vi "Dual Camera Control.vi"(7 "Calling VI Ref":refnum<vi>) -> ()   [LabVIEW 2016]
uses:
  Hardware Configuration/Hardware Configuration Controls/Device Function.ctl
  Dual Camera Control Type Defs/Dual Camera Notifier Type.ctl
  Dual Camera Control Type Defs/Dual Camera Actions.ctl
  <vilib>/Utility/miscctls.llb/LVPointTypeDef.ctl
  Device Library/Cameras/Camera Controls/Generic Camera Actions.ctl
  <vilib>/vision/Image Controls.llb/IMAQ Image.ctl
  Device Library/Cameras/Camera Controls/Generic Camera ROI.ctl
  Hardware Configuration/Hardware Configuration Controls/Device Type.ctl
  Laser Control/Laser Power Control/Laser Power Control Type Defs/Laser Power Ctrl Messenger Actions.ctl
  <vilib>/Utility/error.llb/whitespace.ctl
  shell32.dll
panel:
  in  "Capture":bool
  in  "Preview":bool
  in  "Quit":bool
  out "Current Frame":u32=1
  in  "Exposure Time (s)":dbl=0.1
  in  "Base Save Path":path
  in  "File Name":string="Test Image"
  in  "Number of Frames":u32=1
  in  "Camera 02":bool=TRUE
  in  "Camera 01":bool=TRUE
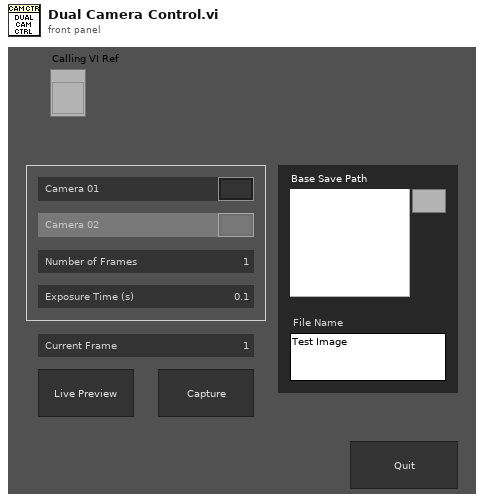
[diagram p1: front panel]
types:
  T1 = typedef "Generic Camera Actions.ctl" = enum16{"Status", "Live Preview", "Capture", "Abort", "Set Exposure Time (s)", "Get Exposure Time (s)", "Record Settings", "Binning", "Set ROI", "Get ROI", "Defect Correction On?", "Cooler On?", "Fan On?", "Quit"}
  T2 = typedef "Generic Camera ROI.ctl" = cluster{"H_Offset":u16, "V_Offset":u16, "H_Width":u16, "V_Width":u16}
  T3 = typedef "IMAQ Image.ctl" = refnum<image>
  T4 = enum16{"Always On", "Always Off", "Off While Running"}
  T5 = typedef "LVPointTypeDef.ctl" = cluster{"Horizontal":i16, "Vertical":i16}
  T6 = typedef "Dual Camera Actions.ctl" = enum16{"Idle", "Exposure Time", "Preview", "Capture", "Set Save Path", "Lasers On", "Lasers Off", "Start Acquisition", "Abort", "Exit Loop", "Quit"}
  T7 = typedef "Dual Camera Notifier Type.ctl" = cluster{"Actions":T6, "Exposure Time (s)":dbl, "Num of Frames":u32, "Save Path":path, "Running?":bool, "Active Cameras":bool[]}
  T8 = typedef "Device Function.ctl" = enum16{"Primary", "Secondary", "Overview", "Wide Field Drift Correction", "642 nm Excitation", "560 nm Excitation", "940 nm Excitation", "546 nm Excitation", "488 nm Excitation", "405 nm Excitation", "Objective Drift Correction", "4Pi Objective Lock", "Objective XY", "Objective Z", "Sample XY", "Sample Coarse Z", "Sample Z", "4Pi Lower", "4Pi Upper", "Mojo", "Adj Cavity", "Line Scanning", "Alert"}
  T9 = enum8{"Enabled", "Disabled", "Disabled and Grayed Out"}
  T10 = typedef "Device Type.ctl" = enum16{"AOTF", "Camera", "Deformable Mirror", "Laser", "Shutter", "Stage", "Waveform", "FPGA", "Email", "Filter Wheel"}
  T11 = typedef "LVRectTypeDef.ctl" = cluster{"Left":i16, "Top":i16, "Right":i16, "Bottom":i16}
  T12 = typedef "LVBoundsTypeDef.ctl" = cluster{"Width":u32, "Height":u32}
  T13 = typedef "Image Type" = u32
  T14 = typedef "whitespace.ctl" = u16
  T15 = typedef "Laser Power Ctrl Messenger Actions.ctl" = enum16{"All Active On", "All Off", "Adjust Power", "Line On/Off", "Get Status"}
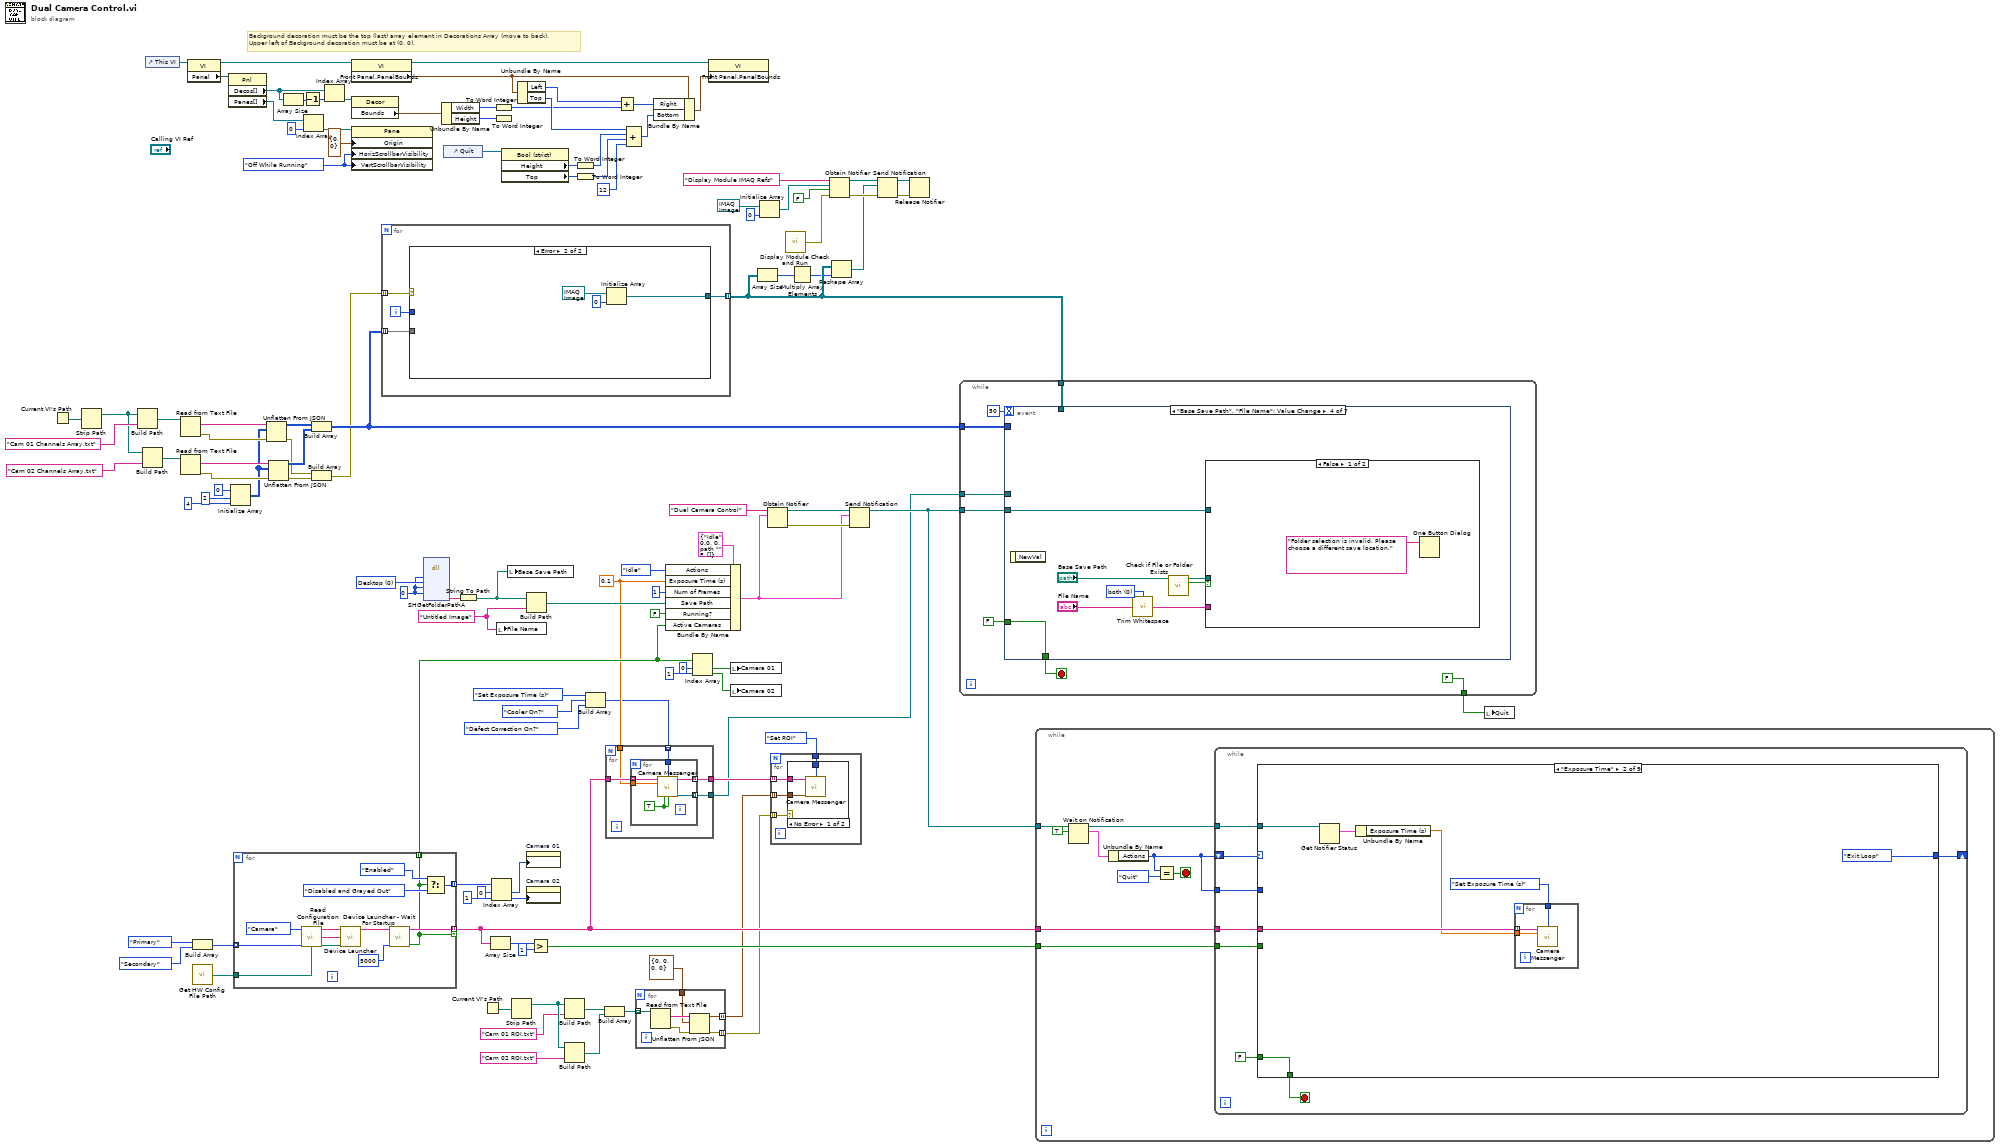
[diagram p0: block diagram]
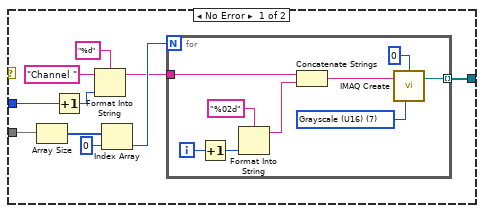
[diagram p3: hidden frame]
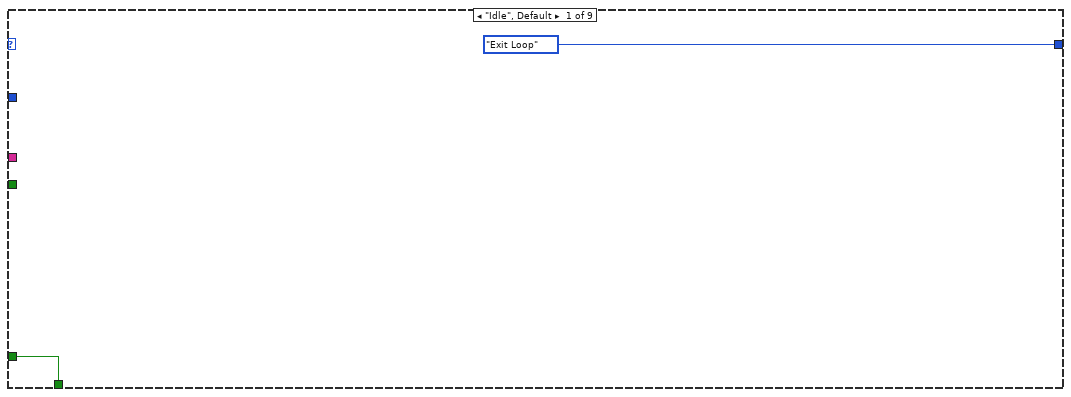
[diagram p4: hidden frame]
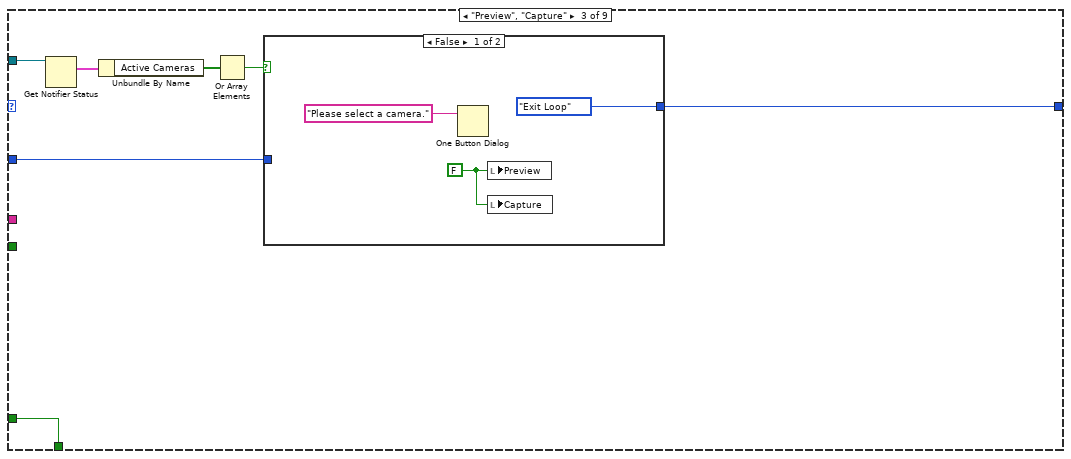
[diagram p5: hidden frame]
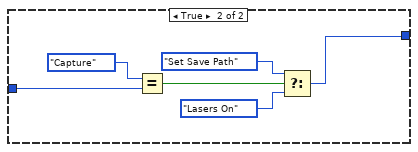
[diagram p6: hidden frame]
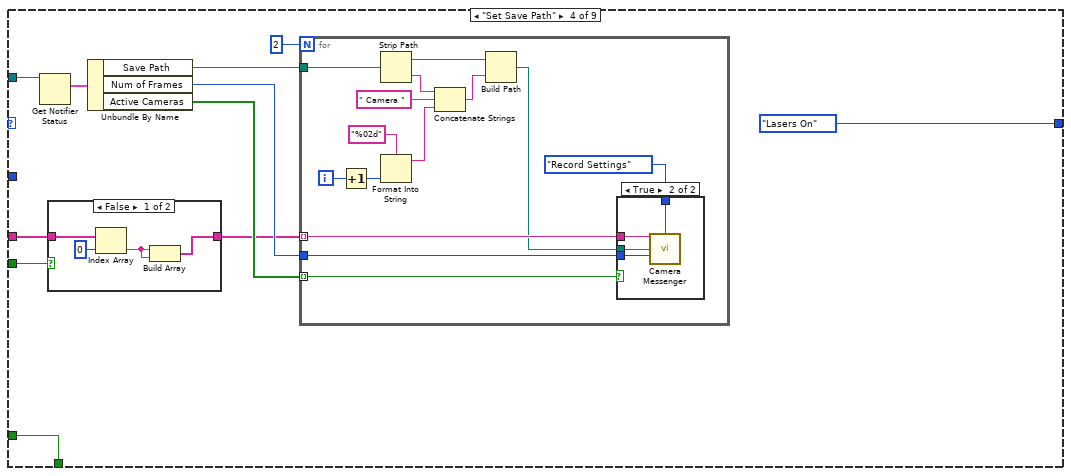
[diagram p7: hidden frame]
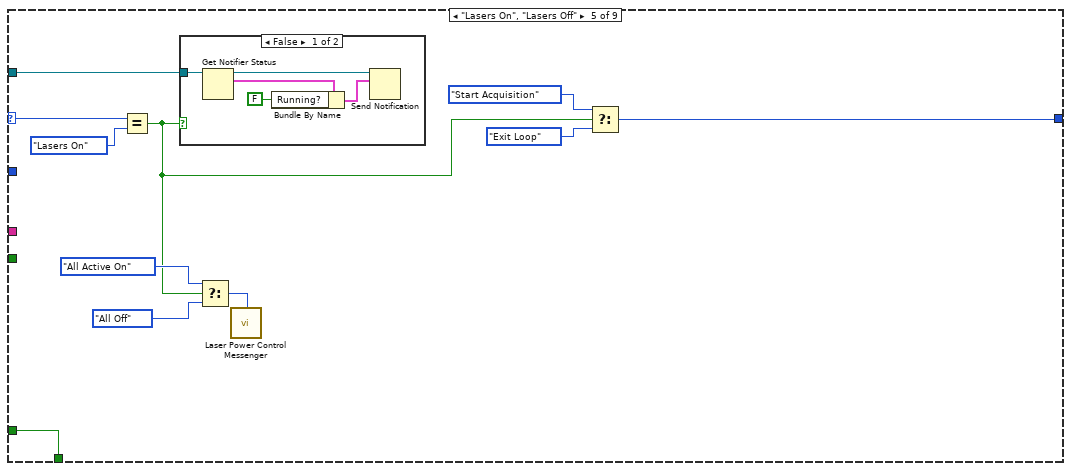
[diagram p10: hidden frame]
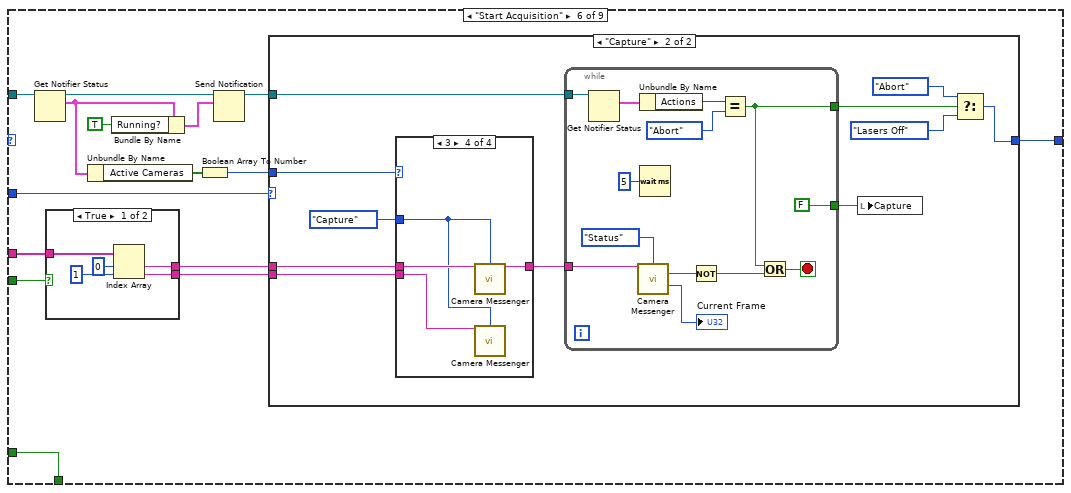
[diagram p12: hidden frame]
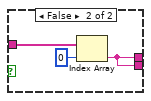
[diagram p13: hidden frame]
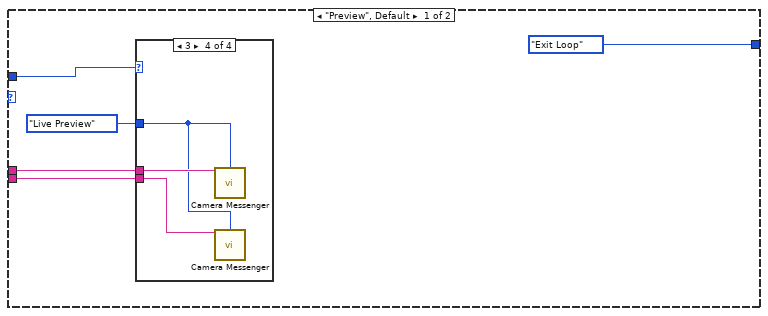
[diagram p14: hidden frame]
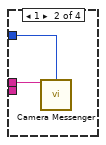
[diagram p16: hidden frame]
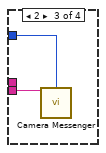
[diagram p17: hidden frame]
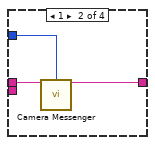
[diagram p19: hidden frame]
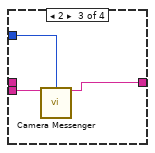
[diagram p20: hidden frame]
diagram:
  w65 = T4."Off While Running" ("Vertical Scrollbar Visibility")
  w39 = 0.1 ("Exposure Time (s)")
  w108 = "Untitled Image"
  w111 = 0 items=["Desktop"=0, "Personal Documents"=5, "AppData"=26, "Local AppData"=28, "Common AppData"=35, "Program Files"=38, "Program Files Common"=43, "Common Documents"=46] ("Requested Path")
  w110 = 0 ("HWND")
  # "Background decoration must be the top (last) array element in Decorations Array (move to back).\nUpper left of Background decoration must be at (0, 0)."
  n1 = Current VI's Path() -> (path=w49:path)
  n2 = Strip Path(path=w49) -> (stripped path=w48:path)  [unwired: 1 out]
  n3 = Build Path(base path=w48, name or relative path="Cam 01 Channels Array.txt") -> (appended path=w52:path)
  n4 = Build Path(base path=w48, name or relative path="Cam 02 Channels Array.txt") -> (appended path=w42:path)
  n5 = control-ref of="This VI"() -> (w57:refnum<vi>)
  n6 = Read from Text File(file (use dialog)=w52) -> (text=w51:string, error out=w50:errorcluster)  [unwired: 3 in, 2 out]
  n7 = Read from Text File(file (use dialog)=w42) -> (text=w45:string, error out=w46:errorcluster)  [unwired: 3 in, 2 out]
  n8 = property class="VI"(reference=w57) -> (reference out=w66:refnum<vi>, "Panel"=w58:refnum<vi>)  [unwired: 1 in, 1 out]
  n9 = Build Array(Device_Function."Primary" ("Device Function"), Device_Function."Secondary" ("Device Function")) -> (w113:T8[])
  n10 = call "Get HW Config File Path.vi"() -> ("File Path"=w96:path)  [unwired: 14 in, 1 out]
  n11 = property class="Pnl"(reference=w58) -> ("Decos[]"=w56:refnum<vi>[], "Panes[]"=w62:refnum<vi>[])  [unwired: 1 in, 2 out]
  n12 = Initialize Array(0 ("element"), 2 ("dimension size"), 4 ("dimension size")) -> (w41:i32[][])
  n13 = for {
    tunnel: w113 -> [w124] mode=indexing
    tunnel: w96 -> [w123]
    tunnel: [w121] -> w40 mode=indexing if=w116
    tunnel: [w117] -> w95 mode=indexing
    tunnel: [w116] -> w87 mode=indexing
    n14 = call "Read Configuration File.vi"("Device Type"=Device_Type."Camera", "Device Function"=w124, "Config File Path"=w123) -> ("Unique Notifier Name"=w126:string, "Device Ports/IDs/Channels"=w128:string[], "Device Engine Path"=w127:path)  [unwired: 9 in, 1 out]
    n15 = call "Device Launcher.vi"("Notifier Name"=w126, "Device Ports/IDs/Channels"=w128, "Device Engine Path"=w127) -> ("Notifier Name"=w122:string)  [unwired: 11 in, 1 out]
    n16 = call "Device Launcher - Wait For Startup.vi"("Notifier Name"=w122, "Wait Time (ms)"=5000) -> ("Notifier Name (Dup)"=w121:string, "Running?"=w116:bool)  [unwired: 12 in]
    n17 = Select(t=T9."Enabled" ("Disabled"), s=w116, f=T9."Disabled and Grayed Out" ("Disabled")) -> (s? t:f=w117:T9)
  }
  n18 = Unflatten From JSON(JSON string=w51, type and defaults=w41, error in (no error)=w50) -> (value=w37:i32[][], error out=w10:errorcluster)  [unwired: 4 in]
  n19 = Unflatten From JSON(JSON string=w45, type and defaults=w41, error in (no error)=w46) -> (value=w38:i32[][], error out=w9:errorcluster)  [unwired: 4 in]
  n20 = Array Size(array=w56) -> (size(s)=w54:i32)
  n21 = Decrement(x=w54) -> (x-1=w55:i32)
  n22 = Index Array(array=w62, index=0) -> (element=w61:refnum<vi>)
  n23 = Build Array(w37, w38) -> (w25:i32[][][])
  n24 = Build Array(w10, w9) -> (w8:errorcluster[])
  n25 = Index Array(array=w56, index=w55) -> (element=w64:refnum<vi>)
  n26 = property class="VI"(reference=w66) -> (reference out=w68:refnum<vi>, "Front Panel.PanelBounds"=w69:T11)  [unwired: 1 in, 1 out]
  n27 = property class="Decor"(reference=w64) -> ("Bounds"=w67:T12)  [unwired: 1 in, 2 out]
  n28 = property class="Pane"(reference=w61, "Origin"=T5 {"Horizontal"=0, "Vertical"=0}, "HorizScrollbarVisibility"=w65, "VertScrollbarVisibility"=w65) -> ()  [unwired: 1 in, 2 out]
  n29 = for {
    tunnel: w25 -> [w132] mode=indexing
    tunnel: [w130] -> w23 mode=indexing
    tunnel: w8 -> [w129] mode=indexing
    i -> [w131]
    n30 = case shown="Error" w129 {
      tunnel: w132 -> [w140 _]
      tunnel: w131 -> [w136 _]
      tunnel: [w133 w152] -> w130
      frame No Error {
        n31 = Array Size(array=w140) -> (size(s)=w142:i32[])
        n32 = Increment(x=w136) -> (x+1=w137:i32)
        n33 = Format Into String(format string="%d", initial string="Channel " ("name (unnamed)"), w137) -> (resulting string=w134:string)  [unwired: 1 in, 1 out]
        n34 = Index Array(array=w142, index=0) -> (element=w139:i32)
        n35 = for {
          N: w139 -> [_]
          tunnel: [w147] -> w133 mode=indexing
          tunnel: w134 -> [w143]
          i -> [w151]
          w150 = T13 7 items=["Grayscale (U8)", "Grayscale (I16)", "Grayscale (SGL)", "Complex (CSG)", "RGB (U32)", "HSL (U32)", "RGB (U64)", "Grayscale (U16)"] ("Image Type")
          n36 = Increment(x=w151) -> (x+1=w145:i32)
          n37 = Format Into String(format string="%02d", w145) -> (resulting string=w144:string)  [unwired: 2 in, 1 out]
          n38 = Concatenate Strings(w143, w144) -> (w148:string)
          n39 = call "IMAQ Create"("Border Size"=0, "Image Name"=w148, "Image Type"=w150) -> ("New Image"=w147:T3)  [unwired: 2 in, 1 out]
        }
      }
      frame Error {
        n40 = Initialize Array(T3 refnum ("New Image"), 0 ("dimension size")) -> (w152:T3[])
      }
    }
  }
  n41 = dll-call lib="shell32.dll" fn="SHGetFolderPathA"("HWND"=w110, "nFolder"=w111, "hToken"=w110, "dwFlags"=w110) -> ("pszPath"=w109:string)  [unwired: 9 in, 2 out]
  n42 = Unbundle By Name(w67) -> ("Width"=w72:u32, "Height"=w75:u32)
  n43 = control-ref of="Quit"() -> (w59:refnum<vi>)
  n44 = String To Path(string=w109) -> (path=w107:path)
  n45 = Current VI's Path() -> (path=w18:path)
  n46 = Array Size(array=w40) -> (size(s)=w90:i32)
  n47 = Index Array(array=w95, index #1=0 ("index"), index #2=1 ("index")) -> (element #1=w91:T9, element #2=w92:T9)
  n48 = To Word Integer(number=w72) -> (16bit integer=w74:i16)
  n49 = To Word Integer(number=w75) -> ()  [unwired: 1 out]
  n50 = local write "File Name"(w108) -> ()
  n51 = property class="Bool (strict)"(reference=w59) -> ("Height"=w77:u32, "Top"=w78:i32)  [unwired: 1 in, 2 out]
  n52 = local write "Base Save Path"(w107) -> ()
  n53 = Strip Path(path=w18) -> (stripped path=w19:path)  [unwired: 1 out]
  n54 = Unbundle By Name(w69) -> ("Left"=w71:i16, "Top"=w82:i16)
  n55 = Build Path(base path=w107, name or relative path=w108) -> (appended path=w103:path)
  n56 = property on="Camera 01" class="Bool (strict)"("DisabledEnum"=w91) -> ()  [unwired: 2 in, 2 out]
  n57 = property on="Camera 02" class="Bool (strict)"("DisabledEnum"=w92) -> ()  [unwired: 2 in, 2 out]
  n58 = Greater?(x=w90, y=1) -> (0:w88:bool)
  n59 = Build Path(base path=w19, name or relative path="Cam 01 ROI.txt") -> (appended path=w14:path)
  n60 = Build Path(base path=w19, name or relative path="Cam 02 ROI.txt") -> (appended path=w13:path)
  n61 = To Word Integer(number=w77) -> (16bit integer=w80:i16)
  n62 = To Word Integer(number=w78) -> (16bit integer=w81:i16)
  n63 = Build Array(Generic_Camera_Actions."Set Exposure Time (s)" ("General Camera Actions"), Generic_Camera_Actions."Cooler On?" ("General Camera Actions"), Generic_Camera_Actions."Defect Correction On?" ("General Camera Actions")) -> (w4:T1[])
  n64 = Build Array(w14, w13) -> (w12:path[])
  n65 = for {
    tunnel: w40 -> [w159]
    tunnel: w39 -> [w158]
    tunnel: [w157] -> w16
    tunnel: w4 -> [w156] mode=indexing
    tunnel: [w155] -> w3
    n66 = for {
      tunnel: w159 -> [w165] mode=indexing
      tunnel: w158 -> [w164]
      tunnel: w156 -> [w163]
      tunnel: [w162] -> w155 mode=indexing
      tunnel: [w161] -> w157 mode=indexing
      w160 = TRUE ("Cooler On/Off")
      n67 = call "Camera Messenger.vi"("Notifier Name"=w165, "General Camera Actions"=w163, "Exposure Time (s)"=w164, "Cooler On?"=w160, "Defect Correction On?"=w160) -> ("Notifier Name Dup"=w161:string, "Image Ref"=w162:T3)  [unwired: 5 in, 4 out]
    }
  }
  n68 = Add(x=w71, y=w74) -> (x+y=w73:i16)
  n69 = Compound Arithmetic op=ADD(w82, w80, w81, i16 12 ("y")) -> (w76:i16)
  n70 = for {
    tunnel: w12 -> [w169] mode=indexing
    tunnel: T2 {"H_Offset"=0, "V_Offset"=0, "H_Width"=0, "V_Width"=0} ("General_Camera_ROI") -> [w168]
    tunnel: [w167] -> w1 mode=indexing
    tunnel: [w166] -> w2 mode=indexing
    n71 = Read from Text File(file (use dialog)=w169) -> (text=w170:string, error out=w171:errorcluster)  [unwired: 3 in, 2 out]
    n72 = Unflatten From JSON(JSON string=w170, type and defaults=w168, error in (no error)=w171) -> (value=w167:T2, error out=w166:errorcluster)  [unwired: 4 in]
  }
  n73 = Bundle By Name(cluster=w69, "Right"=w73, "Bottom"=w76) -> (w70:T11)
  n74 = Bundle By Name(cluster=T7 {"Actions"=enum."Idle", "Exposure Time (s)"=0.0, "Num of Frames"=0, "Save Path"=path "", "Running?"=FALSE, "Active Cameras"=[]} ("Dual Camera Notifier Type"), "Actions"=Dual_Camera_Actions."Idle", "Exposure Time (s)"=w39, "Num of Frames"=u32 1, "Save Path"=w103, "Running?"=FALSE, "Active Cameras"=w87) -> (w99:T7)
  n75 = Index Array(array=w87, index #1=0 ("index"), index #2=1 ("index")) -> (element #1=w84:bool, element #2=w83:bool)
  n76 = property class="VI"(reference=w68, "Front Panel.PanelBounds"=w70) -> ()  [unwired: 1 in, 2 out]
  n77 = local write "Camera 01"(w84) -> ()
  n78 = local write "Camera 02"(w83) -> ()
  n79 = Array Size(array=w23) -> (size(s)=w24:i32[])
  n80 = Initialize Array(T3 refnum ("New Image"), 0 ("dimension size")) -> (w28:T3[])
  n81 = Obtain Notifier(name (unnamed)="Dual Camera Control", notification data type=w99) -> (notifier out=w101:refnum<notifier>, error out=w100:errorcluster)  [unwired: 2 in, 1 out]
  n82 = for {
    tunnel: w16 -> [w175] mode=indexing
    tunnel: Generic_Camera_Actions."Set ROI" ("General Camera Actions") -> [w174]
    tunnel: w2 -> [w173] mode=indexing
    tunnel: w1 -> [w172] mode=indexing
    n83 = case shown="No Error" w173 {
      tunnel: w175 -> [w178 _]
      tunnel: w174 -> [w177 _]
      tunnel: w172 -> [w176 _]
      frame No Error {
        n84 = call "Camera Messenger.vi"("Notifier Name"=w178, "General Camera Actions"=w177, "Camera ROI"=w176) -> ()  [unwired: 7 in, 6 out]
      }
      frame Error {
      }
    }
  }
  n85 = call "Display Module Check and Run.vi"() -> ("Error"=w27:errorcluster)  [unwired: 15 in]
  n86 = Multiply Array Elements(1:w24) -> (0:w22:i32)
  n87 = Obtain Notifier(name (unnamed)="Display Module IMAQ Refs", notification data type=w28, create if not found? (T)=FALSE, error in (no error)=w27) -> (notifier out=w36:refnum<notifier>, error out=w33:errorcluster)  [unwired: 1 out]
  n88 = Reshape Array(w23, w22) -> (w21:T3[])
  n89 = Send Notification(notification=w99, notifier=w101, error in (no error)=w100) -> (notifier out=w97:refnum<notifier>)  [unwired: 1 out]
  n90 = Send Notification(notification=w21, notifier=w36, error in (no error)=w33) -> (notifier out=w35:refnum<notifier>, error out=w34:errorcluster)
  n91 = Release Notifier(notifier=w35, error in (no error)=w34) -> ()  [unwired: 1 in, 3 out]
  n92 = while {
    tunnel: w97 -> [w184]
    tunnel: [FALSE] -> w98
    tunnel: w3 -> [w181]
    tunnel: w25 -> [w182]
    tunnel: w23 -> [w179]
    stop <- w185 stop-if-true
    n93 = event shown="[3] \"Base Save Path\", \"File Name\": Value Change" {
      selector: _ -> [_ _ _ _ _ _ _]
      dyn-events: _ -> [_ _ _ _ _ _ _]
      timeout: 50 -> [_ _ _ _ _ _ _]
      tunnel: FALSE -> [w190 w213 w220 w228 w246 w257 _]
      tunnel: [w190 w213 w220 w228 w246 w257 TRUE] -> w185
      tunnel: w184 -> [_ w212 w219 w227 w245 w256 w261]
      tunnel: w182 -> [w188 _ _ _ _ _ _]
      tunnel: w181 -> [w189 _ _ _ _ _ _]
      tunnel: w179 -> [w187 _ _ _ _ _ _]
      event Timeout {
        n94 = event-data() -> ()  [unwired: 1 in, 3 out]
        n95 = for {
          tunnel: w189 -> [w193] mode=indexing
          tunnel: w188 -> [w192] mode=indexing
          tunnel: w187 -> [w191] mode=indexing
          n96 = call "IMAQ ImageToArray"("Image"=w193) -> ("Image Pixels (U16)"=w194:u16[][])  [unwired: 3 in, 4 out]
          n97 = for {
            tunnel: w191 -> [w205] mode=indexing
            tunnel: w194 -> [w206]
            tunnel: w192 -> [w203] mode=indexing
            n98 = Index Array(array=w203, index #1=0 ("index"), index #2=2 ("index"), index #3=1 ("index"), index #4=3 ("index")) -> (element #1=w201:i32, element #2=w200:i32, element #3=w196:i32, element #4=w195:i32)
            n99 = Array Subset(array=w206, index (row)=w201, length (row)=w200, index (col)=w196, length (col)=w195) -> (w204:u16[][])
            n100 = call "IMAQ ArrayToImage"("Image Pixels (U16)"=w204, "Image"=w205) -> ()  [unwired: 8 in, 2 out]
          }
        }
      }
      event "Exposure Time (s)": Value Change {
        n101 = event-data() -> ("NewVal"=w210:dbl)  [unwired: 1 in]
        n102 = Get Notifier Status(notifier=w212) -> (notifier out=w208:refnum<notifier>, current notification=w211:T7)  [unwired: 1 in, 3 out]
        n103 = Bundle By Name(cluster=w211, "Exposure Time (s)"=w210, "Actions"=Dual_Camera_Actions."Exposure Time") -> (w207:T7)
        n104 = Send Notification(notification=w207, notifier=w208) -> ()  [unwired: 1 in, 2 out]
      }
      event "Number of Frames": Value Change {
        n105 = event-data() -> ("NewVal"=w217:u32)  [unwired: 1 in]
        n106 = Get Notifier Status(notifier=w219) -> (notifier out=w215:refnum<notifier>, current notification=w218:T7)  [unwired: 1 in, 3 out]
        n107 = Bundle By Name(cluster=w218, "Num of Frames"=w217, "Actions"=Dual_Camera_Actions."Idle") -> (w214:T7)
        n108 = Send Notification(notification=w214, notifier=w215) -> ()  [unwired: 1 in, 2 out]
      }
      event "Base Save Path", "File Name": Value Change {
        w224 = T14 0 items=["both", "start of string", "end of string"] ("location (both)")
        n109 = event-data() -> ()  [unwired: 1 in, 1 out]
        n110 = call <vilib>:"Trim Whitespace.vi"("string"="File Name", "location (both)"=w224) -> ("trimmed string"=w225:string)
        n111 = call <vilib>:"Check if File or Folder Exists.vi"("path"="Base Save Path") -> ("file or folder exists?"=w221:bool, "dup path"=w222:path)  [unwired: 8 in, 1 out]
        n112 = case shown="False" w221 {
          tunnel: w227 -> [_ w237]
          tunnel: w225 -> [_ w231]
          tunnel: w222 -> [_ w230]
          frame False {
            n113 = One Button Dialog(message="Folder selection is invalid. Please choose a different save location.") -> ()  [unwired: 1 in, 1 out]
          }
          frame True {
            n114 = Build Path(base path=w230, name or relative path=w231) -> (appended path=w232:path)
            n115 = Get Notifier Status(notifier=w237) -> (notifier out=w235:refnum<notifier>, current notification=w236:T7)  [unwired: 1 in, 3 out]
            n116 = Bundle By Name(cluster=w236, "Actions"=Dual_Camera_Actions."Idle", "Save Path"=w232) -> (w234:T7)
            n117 = Send Notification(notification=w234, notifier=w235) -> ()  [unwired: 1 in, 2 out]
          }
        }
      }
      event "Camera 01", "Camera 02": Value Change {
        n118 = event-data() -> ()  [unwired: 1 in, 1 out]
        n119 = Build Array("Camera 01", "Camera 02") -> (w238:bool[])
        n120 = Get Notifier Status(notifier=w245) -> (notifier out=w243:refnum<notifier>, current notification=w244:T7)  [unwired: 1 in, 3 out]
        n121 = Bundle By Name(cluster=w244, "Actions"=Dual_Camera_Actions."Idle", "Active Cameras"=w238) -> (w242:T7)
        n122 = Send Notification(notification=w242, notifier=w243) -> ()  [unwired: 1 in, 2 out]
      }
      event "Preview", "Capture": Value Change {
        n123 = event-data() -> ("NewVal"=w251:bool, "CtlRef"=w252:refnum<vi>)  [unwired: 1 in]
        n124 = property class="Bool (strict)"(reference=w252) -> ("Label.Text"=w249:string)  [unwired: 1 in, 2 out]
        n125 = case shown="\"Preview\", Default" w249 {
          tunnel: [Dual_Camera_Actions."Preview" ("Actions") Dual_Camera_Actions."Capture" ("Actions")] -> w248
          frame "Preview", Default {
          }
          frame "Capture" {
          }
        }
        n126 = Select(t=w248, s=w251, f=Dual_Camera_Actions."Abort" ("Actions")) -> (s? t:f=w250:T6)
        n127 = Get Notifier Status(notifier=w256) -> (notifier out=w254:refnum<notifier>, current notification=w255:T7)  [unwired: 1 in, 3 out]
        n128 = Bundle By Name(cluster=w255, "Actions"=w250) -> (w253:T7)
        n129 = Send Notification(notification=w253, notifier=w254) -> ()  [unwired: 1 in, 2 out]
      }
      event "Quit": Value Change {
        n130 = event-data() -> ()  [unwired: 1 in, 1 out]
        n131 = Get Notifier Status(notifier=w261) -> (notifier out=w263:refnum<notifier>, current notification=w262:T7)  [unwired: 1 in, 3 out]
        n132 = Bundle By Name(cluster=w262, "Actions"=Dual_Camera_Actions."Quit") -> (w264:T7)
        n133 = Send Notification(notification=w264, notifier=w263) -> ()  [unwired: 1 in, 2 out]
      }
    }
  }
  n134 = while {
    tunnel: w97 -> [w274]
    tunnel: w40 -> [w268]
    tunnel: w88 -> [w266]
    stop <- w270 stop-if-true
    n135 = Wait on Notification(notifier=w274, ignore previous (F)=TRUE) -> (notifier out=w269:refnum<notifier>, notification=w272:T7)  [unwired: 2 in, 2 out]
    n136 = Unbundle By Name(w272) -> ("Actions"=w267:T6)
    n137 = Equal?(x=w267, y=Dual_Camera_Actions."Quit" ("Actions")) -> (x = y?=w270:bool)
    n138 = while {
      shift-right: [w277] -> _
      shift-left: w267 -> [w281]
      tunnel: w269 -> [w282]
      tunnel: w268 -> [w278]
      tunnel: w267 -> [w276]
      tunnel: w266 -> [w275]
      stop <- w279 stop-if-true
      n139 = case shown="\"Exposure Time\"" w281 {
        selector: w281 -> [_ _ _ _ w351 _ _ _ _]
        tunnel: w282 -> [_ w289 w298 w319 w349 w373 w435 _ w446]
        tunnel: FALSE -> [w284 w290 w301 w321 w355 w375 w438 _ _]
        tunnel: [w284 w290 w301 w321 w355 w375 w438 TRUE TRUE] -> w279
        tunnel: w278 -> [_ w288 _ w312 _ w370 w437 _ w445]
        tunnel: [Dual_Camera_Actions."Exit Loop" ("Actions") Dual_Camera_Actions."Exit Loop" ("Actions") w299 Dual_Camera_Actions."Lasers On" ("Actions") w352 w366 Dual_Camera_Actions."Lasers Off" ("Actions") Dual_Camera_Actions."Exit Loop" ("Actions") Dual_Camera_Actions."Quit" ("Actions")] -> w277
        tunnel: w276 -> [_ _ w300 _ _ w374 _ _ _]
        tunnel: w275 -> [_ _ _ w313 _ w367 _ _ _]
        frame "Idle", Default {
        }
        frame "Exposure Time" {
          n140 = Get Notifier Status(notifier=w289) -> (current notification=w287:T7)  [unwired: 1 in, 4 out]
          n141 = Unbundle By Name(w287) -> ("Exposure Time (s)"=w286:dbl)
          n142 = for {
            tunnel: w288 -> [w294] mode=indexing
            tunnel: w286 -> [w293]
            tunnel: Generic_Camera_Actions."Set Exposure Time (s)" ("General Camera Actions") -> [w292]
            n143 = call "Camera Messenger.vi"("Notifier Name"=w294, "General Camera Actions"=w292, "Exposure Time (s)"=w293) -> ()  [unwired: 7 in, 6 out]
          }
        }
        frame "Preview", "Capture" {
          n144 = Get Notifier Status(notifier=w298) -> (current notification=w297:T7)  [unwired: 1 in, 4 out]
          n145 = Unbundle By Name(w297) -> ("Active Cameras"=w296:bool[])
          n146 = Or Array Elements(Boolean array=w296) -> (logical OR=w295:bool)
          n147 = case shown="False" w295 {
            tunnel: w300 -> [_ w310]
            tunnel: [Dual_Camera_Actions."Exit Loop" ("Actions") w305] -> w299
            frame False {
              w302 = FALSE ("Preview")
              n148 = One Button Dialog(message="Please select a camera.") -> ()  [unwired: 1 in, 1 out]
              n149 = local write "Preview"(w302) -> ()
              n150 = local write "Capture"(w302) -> ()
            }
            frame True {
              n151 = Equal?(x=Dual_Camera_Actions."Capture", y=w310) -> (x = y?=w307:bool)
              n152 = Select(t=Dual_Camera_Actions."Set Save Path" ("Actions"), s=w307, f=Dual_Camera_Actions."Lasers On" ("Actions")) -> (s? t:f=w305:T6)
            }
          }
        }
        frame "Set Save Path" {
          n153 = Get Notifier Status(notifier=w319) -> (current notification=w318:T7)  [unwired: 1 in, 4 out]
          n154 = case shown="False" w313 {
            tunnel: w312 -> [w325 w326]
            tunnel: [w322 w326] -> w311
            frame False {
              n155 = Index Array(array=w325, index=0) -> (element=w323:string)
              n156 = Build Array(w323, w323) -> (w322:string[])
            }
            frame True {
            }
          }
          n157 = Unbundle By Name(w318) -> ("Save Path"=w316:path, "Num of Frames"=w317:u32, "Active Cameras"=w315:bool[])
          n158 = for {
            N: 2 -> [_]
            tunnel: w311 -> [w331] mode=indexing
            tunnel: w317 -> [w329]
            tunnel: w316 -> [w332]
            tunnel: w315 -> [w328] mode=indexing
            i -> [w334]
            n159 = Increment(x=w334) -> (x+1=w333:i32)
            n160 = Strip Path(path=w332) -> (stripped path=w337:path, name=w336:string)
            n161 = Format Into String(format string="%02d", w333) -> (resulting string=w335:string)  [unwired: 2 in, 1 out]
            n162 = Concatenate Strings(w336, " Camera " ("string"), w335) -> (w338:string)
            n163 = Build Path(base path=w337, name or relative path=w338) -> (appended path=w330:path)
            n164 = case shown="True" w328 {
              tunnel: w331 -> [_ w344]
              tunnel: w330 -> [_ w343]
              tunnel: w329 -> [_ w342]
              tunnel: Generic_Camera_Actions."Record Settings" ("General Camera Actions") -> [_ w341]
              frame False {
              }
              frame True {
                n165 = call "Camera Messenger.vi"("Notifier Name"=w344, "General Camera Actions"=w341, "Save Path"=w343, "No. of Frames"=w342) -> ()  [unwired: 6 in, 6 out]
              }
            }
          }
        }
        frame "Lasers On", "Lasers Off" {
          n166 = Equal?(x=w351, y=Dual_Camera_Actions."Lasers On" ("x")) -> (x = y?=w346:bool)
          n167 = case shown="False" w346 {
            tunnel: w349 -> [w356 _]
            frame False {
              n168 = Get Notifier Status(notifier=w356) -> (notifier out=w357:refnum<notifier>, current notification=w360:T7)  [unwired: 1 in, 3 out]
              n169 = Bundle By Name(cluster=w360, "Running?"=FALSE) -> (w358:T7)
              n170 = Send Notification(notification=w358, notifier=w357) -> ()  [unwired: 1 in, 2 out]
            }
            frame True {
            }
          }
          n171 = Select(t=Laser_Power_Ctrl_Messenger_Actions."All Active On" ("Power Ctrl Actions"), s=w346, f=Laser_Power_Ctrl_Messenger_Actions."All Off" ("Power Ctrl Actions")) -> (s? t:f=w345:T15)
          n172 = call "Laser Power Control Messenger.vi"("Power Ctrl Actions"=w345) -> ()  [unwired: 13 in, 2 out]
          n173 = Select(t=Dual_Camera_Actions."Start Acquisition" ("x"), s=w346, f=Dual_Camera_Actions."Exit Loop") -> (s? t:f=w352:T6)
        }
        frame "Start Acquisition" {
          n174 = Get Notifier Status(notifier=w373) -> (notifier out=w362:refnum<notifier>, current notification=w361:T7)  [unwired: 1 in, 3 out]
          n175 = case shown="True" w367 {
            tunnel: w370 -> [w380 w383]
            tunnel: [w377 w381] -> w369
            tunnel: [w376 w381] -> w368
            frame True {
              n176 = Index Array(array=w380, index #1=0 ("index"), index #2=1 ("index")) -> (element #1=w377:string, element #2=w376:string)
            }
            frame False {
              n177 = Index Array(array=w383, index=0) -> (element=w381:string)
            }
          }
          n178 = Unbundle By Name(w361) -> ("Active Cameras"=w372:bool[])
          n179 = Bundle By Name(cluster=w361, "Running?"=TRUE) -> (w364:T7)
          n180 = Boolean Array To Number(Boolean array=w372) -> (number=w371:u32)
          n181 = Send Notification(notification=w364, notifier=w362) -> (notifier out=w363:refnum<notifier>)  [unwired: 1 in, 1 out]
          n182 = case shown="\"Capture\"" w374 {
            tunnel: w371 -> [w388 w406]
            tunnel: w369 -> [w387 w405]
            tunnel: w368 -> [w385 w403]
            tunnel: w363 -> [_ w402]
            tunnel: [Dual_Camera_Actions."Exit Loop" ("Actions") w396] -> w366
            frame "Preview", Default {
              n183 = case shown="3" w388 {
                tunnel: w387 -> [_ w390 _ w394]
                tunnel: Generic_Camera_Actions."Live Preview" ("General Camera Actions") -> [_ w389 w392 w393]
                tunnel: w385 -> [_ _ w391 w395]
                frame 0, Default {
                }
                frame 1 {
                  n184 = call "Camera Messenger.vi"("Notifier Name"=w390, "General Camera Actions"=w389) -> ()  [unwired: 8 in, 6 out]
                }
                frame 2 {
                  n185 = call "Camera Messenger.vi"("Notifier Name"=w391, "General Camera Actions"=w392) -> ()  [unwired: 8 in, 6 out]
                }
                frame 3 {
                  n186 = call "Camera Messenger.vi"("Notifier Name"=w394, "General Camera Actions"=w393) -> ()  [unwired: 8 in, 6 out]
                  n187 = call "Camera Messenger.vi"("Notifier Name"=w395, "General Camera Actions"=w393) -> ()  [unwired: 8 in, 6 out]
                }
              }
            }
            frame "Capture" {
              n188 = case shown="3" w406 {
                tunnel: w405 -> [w420 w423 _ w429]
                tunnel: Generic_Camera_Actions."Capture" ("General Camera Actions") -> [_ w422 w426 w428]
                tunnel: w403 -> [_ _ w425 w430]
                tunnel: [w420 w421 w424 w427] -> w401
                frame 0, Default {
                }
                frame 1 {
                  n189 = call "Camera Messenger.vi"("Notifier Name"=w423, "General Camera Actions"=w422) -> ("Notifier Name Dup"=w421:string)  [unwired: 8 in, 5 out]
                }
                frame 2 {
                  n190 = call "Camera Messenger.vi"("Notifier Name"=w425, "General Camera Actions"=w426) -> ("Notifier Name Dup"=w424:string)  [unwired: 8 in, 5 out]
                }
                frame 3 {
                  n191 = call "Camera Messenger.vi"("Notifier Name"=w429, "General Camera Actions"=w428) -> ("Notifier Name Dup"=w427:string)  [unwired: 8 in, 5 out]
                  n192 = call "Camera Messenger.vi"("Notifier Name"=w430, "General Camera Actions"=w428) -> ()  [unwired: 8 in, 6 out]
                }
              }
              n193 = while {
                tunnel: w402 -> [w419]
                tunnel: w401 -> [w415]
                tunnel: [FALSE] -> w400
                tunnel: [w407] -> w399
                stop <- w411 stop-if-true
                n194 = Get Notifier Status(notifier=w419) -> (current notification=w418:T7)  [unwired: 1 in, 4 out]
                n195 = call "Camera Messenger.vi"("Notifier Name"=w415, "General Camera Actions"=Generic_Camera_Actions."Status") -> ("Running?"=w413:bool, "Current Frame"=→"Current Frame":u32)  [unwired: 8 in, 4 out]
                n196 = Unbundle By Name(w418) -> ("Actions"=w417:T6)
                n197 = Wait (ms)(milliseconds to wait=u32 5) -> ()  [unwired: 1 out]
                n198 = Not(x=w413) -> (.not. x?=w412:bool)
                n199 = Equal?(x=w417, y=Dual_Camera_Actions."Abort") -> (x = y?=w407:bool)
                n200 = Or(x=w407, y=w412) -> (x .or. y?=w411:bool)
              }
              n201 = local write "Capture"(w400) -> ()
              n202 = Select(t=Dual_Camera_Actions."Abort" ("Actions"), s=w399, f=Dual_Camera_Actions."Lasers Off" ("Actions")) -> (s? t:f=w396:T6)
            }
          }
        }
        frame "Abort" {
          n203 = Get Notifier Status(notifier=w435) -> (notifier out=w431:refnum<notifier>, current notification=w434:T7)  [unwired: 1 in, 3 out]
          n204 = for {
            tunnel: w437 -> [w440] mode=indexing
            n205 = call "Camera Messenger.vi"("Notifier Name"=w440, "General Camera Actions"=Generic_Camera_Actions."Abort") -> ()  [unwired: 8 in, 6 out]
          }
          n206 = Bundle By Name(cluster=w434, "Running?"=FALSE) -> (w432:T7)
          n207 = Send Notification(notification=w432, notifier=w431) -> ()  [unwired: 1 in, 2 out]
        }
        frame "Exit Loop" {
        }
        frame "Quit" {
          n208 = Release Notifier(notifier=w446) -> ()  [unwired: 2 in, 3 out]
          n209 = for {
            tunnel: w445 -> [w448] mode=indexing
            n210 = call "Camera Messenger.vi"("Notifier Name"=w448, "General Camera Actions"=Generic_Camera_Actions."Abort") -> ()  [unwired: 8 in, 6 out]
          }
        }
      }
    }
  }
  n211 = local write "Quit"(w98) -> ()
